vi "Server Access Settings.vi"(7 "write? (T)":bool=TRUE, 8 "error in":errorcluster, 9 "Access token":string, 10 "Allowed clients":string[](array[string]), 11 "id":i32) -> (0 "error out":errorcluster, 1 "this computer":string[](array[string]), 2 "access token out":string, 3 "allowed clients out":string[](array[string]))   [LabVIEW 2020, in "MCP Server.lvlib"]
doc: "Functional global that keeps the access settings of every MCP server in this LabVIEW, keyed by server id: the allowed clients and the access token given to Start.vi. Start.vi writes them when it creates a server, before the HTTP server is opened; Check Client Access.vi reads them for every request; Stop.vi clears them by writing an empty token and an empty list for the id. A later write for the same id replaces the earlier one.\n\nthis computer: the names that mean \"this computer\", all in lower case: the computer's full name (FQDN) and its short name as LabVIEW reports them, and its IP address. They are looked up once, on a write, because the lookup can be slow. Check Client Access.vi no longer uses them: it decides \"this computer only\" from the connection's local address.\n\nwrite? (T) TRUE stores Allowed clients and Access token for id; FALSE only reads. The outputs are the stored values for id after the call (empty when nothing is stored for id). The token is stored only here and never logged."
uses:
  MCP Server.lvlib
  8101b8e9-49ee-472e-bcf6-751deb51bf5a.vi
  fb3f592d-3f10-494c-8117-afcfcdd669c9.vi
  <vilib>/JDP Science/JSONtext/Variant to JSON Text.vi
  <vilib>/JDP Science/JSONtext/JSON text to Variant.vi
  <vilib>/JDP Science/JSONtext/LVClass Serializer/JSONtext LVClass Serializer.lvclass
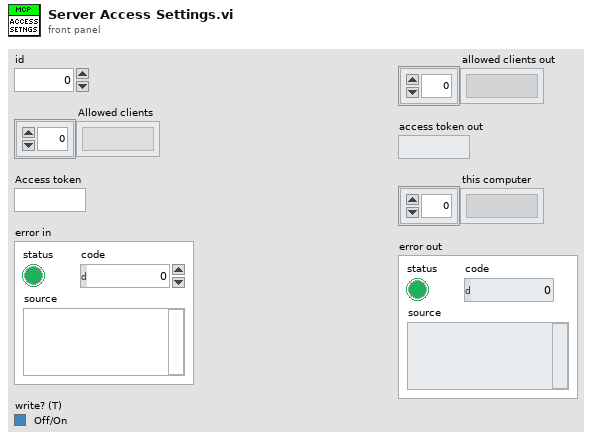
[diagram p1: front panel]
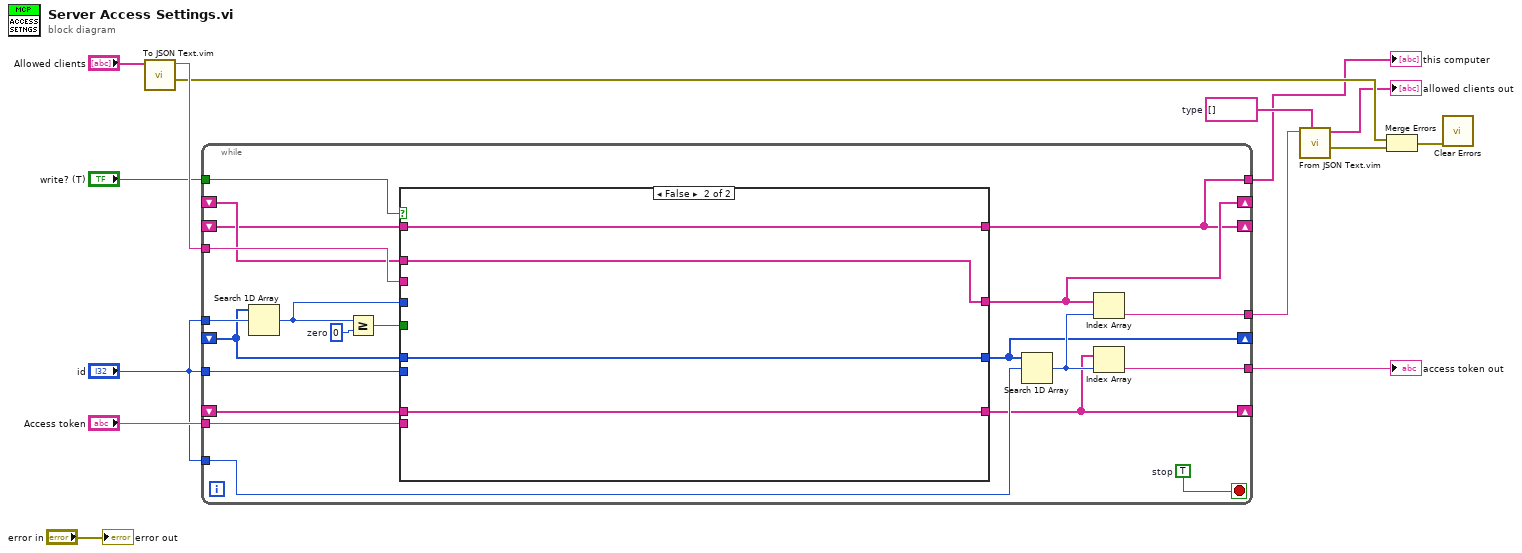
[diagram p0: block diagram]
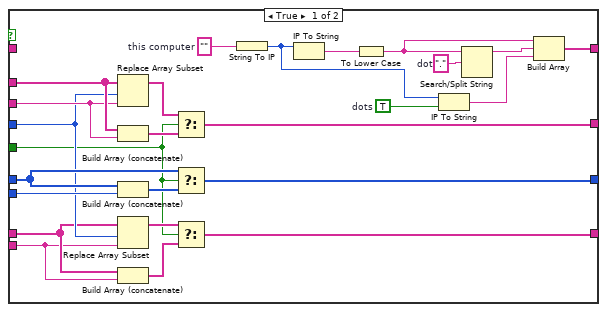
[diagram p2: hidden frame]
diagram:
  w8 = string[] []  # type
  n1 = call "To JSON Text.vim"("Anything"="Allowed clients") -> ("error out"=w7:errorcluster, "<JSON>"=w13:string)  [unwired: 9 in]
  n2 = while {
    tunnel: "id" -> [w35]
    tunnel: "id" -> [w33]
    tunnel: w13 -> [w32]
    tunnel: "Access token" -> [w31]
    tunnel: "write? (T)" -> [w28]
    tunnel: "id" -> [w27]
    shift-right: [w25] -> _
    shift-left: _ -> [w24]
    shift-right: [w23] -> _
    shift-left: _ -> [w22]
    shift-right: [w21] -> _
    shift-left: _ -> [w20]
    shift-right: [w15] -> _
    shift-left: _ -> [w19]
    tunnel: [w17] -> w9
    tunnel: [w16] -> w3
    tunnel: [w15] -> w2
    stop <- w18 stop-if-true
    w18 = TRUE  # stop
    w34 = 0  # zero
    n3 = Search 1D Array(1D array=w24, element=w35) -> (index of element=w30:i32)  [unwired: 1 in]
    n4 = Greater Or Equal?(x=w30, y=w34) -> (x >= y?=w29:bool)
    n5 = case shown="False" w28 {
      tunnel: w24 -> [w59 w64]
      tunnel: w22 -> [w57 w63]
      tunnel: w20 -> [w52 w62]
      tunnel: w19 -> [_ w61]
      tunnel: w33 -> [w60 _]
      tunnel: w32 -> [w56 _]
      tunnel: w31 -> [w51 _]
      tunnel: w30 -> [w53 _]
      tunnel: w29 -> [w49 _]
      tunnel: [w39 w64] -> w25
      tunnel: [w38 w63] -> w23
      tunnel: [w37 w62] -> w21
      tunnel: [w36 w61] -> w15
      frame True {
        w43 = "."  # dot
        w44 = TRUE  # dots
        w47 = ""  # this computer
        n6 = Replace Array Subset(array=w57, new element=w56, index=w53) -> (w55:string[])
        n7 = Build Array (concatenate)(w57, w56) -> (w54:string[])
        n8 = Build Array (concatenate)(w59, w60) -> (w58:i32[])
        n9 = Replace Array Subset(array=w52, new element=w51, index=w53) -> (w50:string[])
        n10 = Build Array (concatenate)(w52, w51) -> (w48:string[])
        n11 = Select(t=w55, s=w49, f=w54) -> (s? t:f=w38:string[])
        n12 = Select(t=w59, s=w49, f=w58) -> (s? t:f=w39:i32[])
        n13 = Select(t=w50, s=w49, f=w48) -> (s? t:f=w37:string[])
        n14 = String To IP(1:w47) -> (0:w45:u32)
        n15 = IP To String(2:w45) -> (0:w46:string)  [unwired: 1 in]
        n16 = To Lower Case(string=w46) -> (all lower case string=w42:string)
        n17 = IP To String(1:w44, 2:w45) -> (0:w40:string)
        n18 = Search/Split String(string=w42, search string/char (-)=w43) -> (substring before match=w41:string)  [unwired: 1 in, 2 out]
        n19 = Build Array(w42, w41, w40) -> (w36:string[])
      }
      frame False {
      }
    }
    n20 = Search 1D Array(1D array=w25, element=w27) -> (index of element=w26:i32)  [unwired: 1 in]
    n21 = Index Array(array=w23, index=w26) -> (element=w17:string)
    n22 = Index Array(array=w21, index=w26) -> (element=w16:string)
  }
  "access token out" <- w3
  "this computer" <- w2
  n23 = call "From JSON Text.vim"("Data Type and Default Value"=w8, "JSON"=w9) -> ("error out"=w6:errorcluster, "Data out"=→"allowed clients out":string[])  [unwired: 8 in]
  n24 = Merge Errors(w7, w6) -> (w5:errorcluster)
  n25 = call <vilib>:"Clear Errors.vi"("error in (no error)"=w5) -> ()  [unwired: 5 in, 2 out]
  "error out" <- "error in"
